vi "RemoteVI Overlay Encode.vi"(0 "popups":cluster{"x":i16, "y":i16, "png":string}[](array[cluster])) -> (4 "message":string)   [LabVIEW 2020, in "RemoteVI.lvlib"]
doc: "Encodes one RemoteVI protocol v2 OVERLAY message (docs/protocol.md section 3.2): the LabVIEW popups open over the panel. Layout, all integers big-endian: 0x52, 0x02, popup count U16, then per popup x I16, y I16, png length U32 and the png bytes - the same record layout as FRAME rects. x and y are relative to the frame origin (the top-left of what the FRAME shows) and may lie outside the frame. An empty popups array gives the 4-byte message that clears the overlay. Pure function, cannot fail. Reference: encodeOverlay() in tools\\lib\\protocol.mjs, vectors tests\\vectors\\frame.json overlays."
uses:
  RemoteVI.lvlib
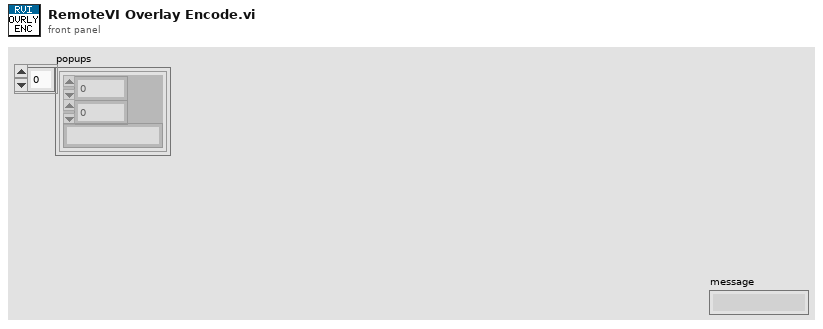
[diagram p1: front panel]
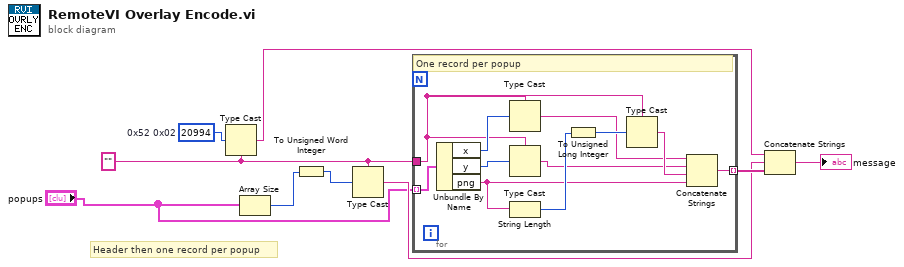
[diagram p0: block diagram]
diagram:
  w3 = ""
  w2 = u16 20994  # 0x52 0x02
  # "Header then one record per popup"
  n1 = Type Cast(type=w3, x=w2) -> (*(type *) &x=w4:string)
  n2 = Array Size(array="popups") -> (size(s)=w5:i32)
  n3 = To Unsigned Word Integer(number=w5) -> (unsigned 16bit integer=w6:u16)
  n4 = Type Cast(type=w3, x=w6) -> (*(type *) &x=w7:string)
  n5 = for {
    tunnel: "popups" -> [w10] mode=indexing
    tunnel: w3 -> [w11]
    tunnel: [w20] -> w8 mode=indexing
    # "One record per popup"
    n6 = Unbundle By Name(w10) -> ("x"=w12:i16, "y"=w13:i16, "png"=w14:string)
    n7 = Type Cast(type=w11, x=w12) -> (*(type *) &x=w15:string)
    n8 = Type Cast(type=w11, x=w13) -> (*(type *) &x=w16:string)
    n9 = String Length(string=w14) -> (length=w17:i32)
    n10 = To Unsigned Long Integer(number=w17) -> (unsigned 32bit integer=w18:u32)
    n11 = Type Cast(type=w11, x=w18) -> (*(type *) &x=w19:string)
    n12 = Concatenate Strings(w15, w16, w19, w14) -> (w20:string)
  }
  n13 = Concatenate Strings(w4, w7, w8) -> (→"message":string)
